vi "test_PhotonPoseEstimator_ClosestToLastfPose.vi"(8 "error in (no error)":errorcluster) -> (0 "error out":errorcluster, 3 "Test Passed":bool)   [LabVIEW 2019]
uses:
  <vilib>/Rock Robotics/WPI/ThirdParty/PhotonVisionLib/TypeDef/PhotonEstimatedRobotPoseType.ctl
  <vilib>/Rock Robotics/WPI/ThirdParty/JAS_Junk/TrajLib/TypeDef/POSE3D.ctl
  <vilib>/Rock Robotics/WPI/ThirdParty/JAS_Junk/TrajLib/TypeDef/TRANSLATION3D.ctl
  <vilib>/Rock Robotics/WPI/ThirdParty/JAS_Junk/TrajLib/TypeDef/ROTATION3D.ctl
  <vilib>/Rock Robotics/WPI/ThirdParty/JAS_Junk/TrajLib/TypeDef/QUATERNION.ctl
  <vilib>/Rock Robotics/WPI/ThirdParty/PhotonVisionLib/TypeDef/PhotonTrackedTargetType.ctl
  <vilib>/Rock Robotics/WPI/ThirdParty/PhotonVisionLib/TypeDef/TargetCornerType.ctl
  <vilib>/Rock Robotics/WPI/ThirdParty/JAS_Junk/TrajLib/TypeDef/TRANSFORM3D.ctl
  <vilib>/Rock Robotics/WPI/ThirdParty/PhotonVisionLib/Enum/PhotonPoseStrategy_ENUM.ctl
  <vilib>/Rock Robotics/WPI/ThirdParty/JAS_Junk/TrajLib/VI/Quaternion_New.vi
  <vilib>/Rock Robotics/WPI/ThirdParty/PhotonVisionLib/SubVI/PhotonTargetModel_New_AprilTag36H11.vi
  <vilib>/Rock Robotics/WPI/ThirdParty/JAS_Junk/TrajLib/VI/TimeInterpRotation2d_New.vi
  <vilib>/Rock Robotics/WPI/ThirdParty/JAS_Junk/TrajLib/VI/Transform3d_Equals.vi
  <vilib>/Rock Robotics/WPI/ThirdParty/PhotonVisionLib/SubVI/PhotonPoseEstimator_SetCamera.vi
  <vilib>/Rock Robotics/WPI/ThirdParty/PhotonVisionLib/SubVI/PhotonPoseEstimator_SetRobotToCameraTransform.vi
  <vilib>/Rock Robotics/WPI/ThirdParty/PhotonVisionLib/SubVI/PhotonEstimatedRobotPose_GetAll.vi
  <vilib>/Rock Robotics/WPI/ThirdParty/JAS_Junk/TrajLib/VI/Pose3d_ToPose2d.vi
  <vilib>/Rock Robotics/WPI/ThirdParty/PhotonVisionLib/SubVI/PhotonPoseEstimator_Update_All.vi
  <vilib>/Rock Robotics/WPI/ThirdParty/PhotonVisionLib/SubVI/PhotonPoseEstimator_GetEmptyPose.vi
  <vilib>/Rock Robotics/WPI/ThirdParty/PhotonVisionLib/SubVI/PhotonPoseEstimator_EstimateClosestToLastPose.vi
  <vilib>/Rock Robotics/WPI/ThirdParty/PhotonVisionLib/SubVI/PhotonPoseEstimator_GetLastPose.vi
  <vilib>/Rock Robotics/WPI/ThirdParty/PhotonVisionLib/SubVI/PhotonPipelineResult_GetTimeStampSecs.vi
  <vilib>/Rock Robotics/WPI/ThirdParty/PhotonVisionLib/SubVI/PhotonTargetModel_New_RectPlanar.vi
  <vilib>/Rock Robotics/WPI/ThirdParty/JAS_Junk/TrajLib/Conv_Inches_Meters.vi
  <vilib>/Rock Robotics/WPI/ThirdParty/JAS_Junk/TrajLib/VI/Transform3d_GetTranslation3d.vi
  <vilib>/Rock Robotics/WPI/ThirdParty/JAS_Junk/TrajLib/VI/Transform3d_GetRotation3d.vi
  <vilib>/Rock Robotics/WPI/ThirdParty/JAS_Junk/TrajLib/VI/Rotation3d_Equals.vi
  <vilib>/Rock Robotics/WPI/ThirdParty/JAS_Junk/TrajLib/VI/Translation3d_Equals.vi
  <vilib>/Rock Robotics/WPI/ThirdParty/JAS_Junk/TrajLib/VI/Pose3d_getTranslation3d.vi
  <vilib>/Rock Robotics/WPI/ThirdParty/JAS_Junk/TrajLib/VI/Pose3d_getRotation3d.vi
  <vilib>/Rock Robotics/WPI/ThirdParty/JAS_Junk/TrajLib/VI/Translation3d_ToTranslation2d.vi
  <vilib>/Rock Robotics/WPI/ThirdParty/JAS_Junk/TrajLib/VI/Rotation3d_ToRotation2d.vi
  <vilib>/Rock Robotics/WPI/ThirdParty/JAS_Junk/TrajLib/Pose2d_New_TRRO.vi
  <vilib>/Rock Robotics/WPI/ThirdParty/PhotonVisionLib/SubVI/PhotonPoseEstimator_EstimateLowestAmbiguityPose.vi
  <vilib>/Rock Robotics/WPI/ThirdParty/PhotonVisionLib/SubVI/PhotonPoseEstimator_EstimateClosestToCameraHeightPose.vi
  <vilib>/Rock Robotics/WPI/ThirdParty/PhotonVisionLib/SubVI/PhotonPoseEstimator_EstimateClosestToReferencePose.vi
  <vilib>/Rock Robotics/WPI/ThirdParty/PhotonVisionLib/SubVI/PhotonPoseEstimator_GetReferencePose.vi
  <vilib>/Rock Robotics/WPI/ThirdParty/PhotonVisionLib/SubVI/PhotonPoseEstimator_SetReferencePose.vi
  <vilib>/Rock Robotics/WPI/ThirdParty/PhotonVisionLib/SubVI/PhotonPoseEstimator_EstimateAverageBestTargetsPose.vi
  <vilib>/Rock Robotics/WPI/ThirdParty/PhotonVisionLib/SubVI/PhotonPoseEstimator_EstimateMultiTagOnCoprocPose.vi
  <vilib>/Rock Robotics/WPI/ThirdParty/PhotonVisionLib/SubVI/PhotonPoseEstimator_EstimatePnpDistanceTrigSolvePose.vi
  <vilib>/Rock Robotics/WPI/ThirdParty/PhotonVisionLib/SubVI/PhotonPoseEstimator_Strategy_constrainedPnpStrategy.vi
  <vilib>/Rock Robotics/WPI/ThirdParty/JAS_Junk/TrajLib/VI/Rotation3d_Create_AxisAngle.vi
  <vilib>/Rock Robotics/WPI/ThirdParty/JAS_Junk/TrajLib/VI/Pose3d_New.vi
  <vilib>/Rock Robotics/WPI/ThirdParty/PhotonVisionLib/SubVI/PhotonPipelineResult_HasTargets.vi
  <vilib>/Rock Robotics/WPI/ThirdParty/PhotonVisionLib/SubVI/PhotonEstimatedRobotPose_New.vi
  <vilib>/Rock Robotics/WPI/ThirdParty/PhotonVisionLib/SubVI/PhotonPipelineResult_GetTargets.vi
  <vilib>/Rock Robotics/WPI/ThirdParty/JAS_Junk/TrajLib/VI/AprilTagFieldLayout_GetTagPose.vi
  <vilib>/Rock Robotics/WPI/ThirdParty/PhotonVisionLib/SubVI/PhotonTrackedTarget_GetFiducialId.vi
  <vilib>/Rock Robotics/WPI/ThirdParty/PhotonVisionLib/SubVI/PhotonTrackedTarget_GetAltCameraToTarget.vi
  <vilib>/Rock Robotics/WPI/ThirdParty/PhotonVisionLib/SubVI/PhotonTrackedTarget_GetBestCameraToTarget.vi
  <vilib>/Rock Robotics/WPI/ThirdParty/PhotonVisionLib/SubVI/PhotonPoseEstimator_Strategy_closestToReferencePose_calc.vi
  <vilib>/Rock Robotics/WPI/ThirdParty/PhotonVisionLib/SubVI/PhotonTrackedTarget_GetPoseAmbiguity.vi
  <vilib>/Rock Robotics/WPI/ThirdParty/PhotonVisionLib/SubVI/PhotonPoseEstimator_GetFieldTags.vi
  <vilib>/Rock Robotics/WPI/ThirdParty/PhotonVisionLib/SubVI/PhotonPoseEstimator_GetRobotToCameraTransform.vi
  <vilib>/Rock Robotics/WPI/ThirdParty/PhotonVisionLib/SubVI/PhotonPoseEstimator_GetHighestAmbiguity.vi
  <vilib>/Rock Robotics/WPI/ThirdParty/PhotonVisionLib/SubVI/PhotonTargetModel_New.vi
  <vilib>/Rock Robotics/WPI/ThirdParty/JAS_Junk/TrajLib/VI/Rotation3d_GetQuaterion.vi
  <vilib>/Rock Robotics/WPI/ThirdParty/JAS_Junk/TrajLib/VI/Quaternion_Equals.vi
  <vilib>/Rock Robotics/WPI/ThirdParty/JAS_Junk/TrajLib/Translation2d_Create.vi
  <vilib>/Rock Robotics/WPI/ThirdParty/JAS_Junk/TrajLib/Rotation2d_CreateAngle.vi
  <vilib>/Rock Robotics/WPI/ThirdParty/JAS_Junk/TrajLib/VI/Rotation3d_GetXYZ.vi
  <vilib>/Rock Robotics/WPI/ThirdParty/JAS_Junk/TrajLib/VI/Pose3d_TransformBy.vi
  <vilib>/Rock Robotics/WPI/ThirdParty/JAS_Junk/TrajLib/VI/Transform3d_Inverse.vi
  <vilib>/Rock Robotics/WPI/ThirdParty/PhotonVisionLib/SubVI/PhotonPoseEstimator_Strategy_closestToCameraHeight_calc.vi
  <vilib>/Rock Robotics/WPI/ThirdParty/PhotonVisionLib/SubVI/PhotonPoseEstimator_Strategy_averageBestTargets_calc.vi
  <vilib>/Rock Robotics/WPI/ThirdParty/JAS_Junk/TrajLib/VI/Rotation3d_Plus.vi
  <vilib>/Rock Robotics/WPI/ThirdParty/JAS_Junk/TrajLib/VI/Translation3d_Plus.vi
  <vilib>/Rock Robotics/WPI/ThirdParty/JAS_Junk/TrajLib/VI/Translation3d_Times.vi
  <vilib>/Rock Robotics/WPI/ThirdParty/JAS_Junk/TrajLib/VI/Rotation3d_Times.vi
  <vilib>/Rock Robotics/WPI/ThirdParty/JAS_Junk/TrajLib/VI/Rotation3d_Create_Default.vi
  <vilib>/Rock Robotics/WPI/ThirdParty/JAS_Junk/TrajLib/VI/Translation3d_Create_Default.vi
  <vilib>/Rock Robotics/WPI/ThirdParty/JAS_Junk/TrajLib/VI/Pose3d_New_Default.vi
  <vilib>/Rock Robotics/WPI/ThirdParty/JAS_Junk/TrajLib/VI/Pose3d_Plus.vi
  <vilib>/Rock Robotics/WPI/ThirdParty/JAS_Junk/TrajLib/VI/Pose3d_RelativeTo.vi
  <vilib>/Rock Robotics/WPI/ThirdParty/JAS_Junk/TrajLib/VI/AprilTagFieldLayout_GetOriginPosition.vi
  <vilib>/Rock Robotics/WPI/ThirdParty/PhotonVisionLib/SubVI/PhotonPipelineResult_GetMultiTagResult.vi
  <vilib>/Rock Robotics/WPI/ThirdParty/PhotonVisionLib/SubVI/PhotonPipelineResult_GetBestTarget.vi
  <vilib>/Rock Robotics/WPI/ThirdParty/PhotonVisionLib/SubVI/PhotonTrackedTarget_GetPitch.vi
  <vilib>/Rock Robotics/WPI/ThirdParty/PhotonVisionLib/SubVI/PhotonTrackedTarget_GetYaw.vi
  <vilib>/Rock Robotics/WPI/ThirdParty/JAS_Junk/TrajLib/Units_DegreesToRadians.vi
  <vilib>/Rock Robotics/WPI/ThirdParty/JAS_Junk/TrajLib/VI/Translation3d_GetNorm.vi
  <vilib>/Rock Robotics/WPI/ThirdParty/JAS_Junk/TrajLib/VI/Translation3d_Create_DistAng.vi
  <vilib>/Rock Robotics/WPI/ThirdParty/JAS_Junk/TrajLib/VI/Translation3d_RotateBy.vi
  <vilib>/Rock Robotics/WPI/ThirdParty/JAS_Junk/TrajLib/Translation2d_RotateBy.vi
  <vilib>/Rock Robotics/WPI/ThirdParty/JAS_Junk/TrajLib/Pose2d_getTranslation.vi
  <vilib>/Rock Robotics/WPI/ThirdParty/JAS_Junk/TrajLib/Translation2d_Plus.vi
  <vilib>/Rock Robotics/WPI/ThirdParty/JAS_Junk/TrajLib/Translation2d_UnaryMinus.vi
  <vilib>/Rock Robotics/WPI/ThirdParty/JAS_Junk/TrajLib/VI/Pose3d_New_Pose2d.vi
  <vilib>/Rock Robotics/WPI/ThirdParty/JAS_Junk/TrajLib/VI/TimeInterpRotation2d_GetSample.vi
  <vilib>/Rock Robotics/WPI/ThirdParty/PhotonVisionLib/SubVI/PhotonPoseEstimator_GetHeadingBuffer.vi
  <vilib>/Rock Robotics/WPI/ThirdParty/JAS_Junk/TrajLib/VI/Vector_Norm.vi
  <vilib>/Rock Robotics/WPI/ThirdParty/JAS_Junk/TrajLib/VecBuilder_ArrayBy1Fill.vi
  <vilib>/Rock Robotics/WPI/ThirdParty/JAS_Junk/TrajLib/VI/AprilTag_GetAll.vi
  <vilib>/Rock Robotics/WPI/ThirdParty/JAS_Junk/TrajLib/Transform2d_Create_TransRot.vi
  <vilib>/Rock Robotics/WPI/ThirdParty/PhotonVisionLib/SubVI/PhotonPoseEstimator_CalcDifference.vi
  <vilib>/Rock Robotics/WPI/ThirdParty/JAS_Junk/TrajLib/VI/Quaternion_Get_Vect.vi
  <vilib>/Rock Robotics/WPI/ThirdParty/JAS_Junk/TrajLib/VI/Quaternion_Get_W.vi
  <vilib>/Rock Robotics/WPI/ThirdParty/JAS_Junk/TrajLib/VI/Quaternion_Get_All.vi
  <vilib>/Rock Robotics/WPI/ThirdParty/JAS_Junk/TrajLib/VI/Rotation3d_UnaryMinus.vi
  <vilib>/Rock Robotics/WPI/ThirdParty/JAS_Junk/TrajLib/VI/Translation3d_UnaryMinus.vi
  <vilib>/Rock Robotics/WPI/ThirdParty/JAS_Junk/TrajLib/VI/Transform3d_GetXYZ.vi
  <vilib>/Rock Robotics/WPI/ThirdParty/JAS_Junk/TrajLib/VI/Pose3d_getXYZ.vi
  <vilib>/Rock Robotics/WPI/ThirdParty/JAS_Junk/TrajLib/VI/Rotation3d_RotateBy.vi
  <vilib>/Rock Robotics/WPI/ThirdParty/JAS_Junk/TrajLib/VI/Translation3d_GetXYZ.vi
  <vilib>/Rock Robotics/WPI/ThirdParty/JAS_Junk/TrajLib/VI/Quaternion_New_Default.vi
  <vilib>/Rock Robotics/WPI/ThirdParty/JAS_Junk/TrajLib/VI/Transform3d_Create_Pose3dPose3d.vi
  <vilib>/Rock Robotics/WPI/ThirdParty/JAS_Junk/TrajLib/Conv_Deg_Radians.vi
  <vilib>/Rock Robotics/WPI/ThirdParty/JAS_Junk/TrajLib/VI/Quaternion_Times.vi
  <vilib>/Rock Robotics/WPI/ThirdParty/JAS_Junk/TrajLib/VI/Quaternion_Inverse.vi
  <vilib>/Rock Robotics/WPI/ThirdParty/JAS_Junk/TrajLib/Pose2d_getXYAngle.vi
  <vilib>/Rock Robotics/WPI/ThirdParty/JAS_Junk/TrajLib/Rotation2d_Interpolate.vi
  <vilib>/Rock Robotics/WPI/ThirdParty/JAS_Junk/TrajLib/MatBuilder_Create.vi
  <vilib>/Rock Robotics/WPI/ThirdParty/JAS_Junk/TrajLib/VI/Translation3d_GetDistance.vi
  <vilib>/Rock Robotics/WPI/ThirdParty/JAS_Junk/TrajLib/VI/Rotation3d_Create_Quaternion.vi
  <vilib>/Rock Robotics/WPI/ThirdParty/JAS_Junk/TrajLib/VI/Translation3d_Minus.vi
  <vilib>/Rock Robotics/WPI/ThirdParty/JAS_Junk/TrajLib/VI/Rotation3d_Minus.vi
  <vilib>/Rock Robotics/WPI/ThirdParty/JAS_Junk/TrajLib/Rotation2d_Plus.vi
  <vilib>/Rock Robotics/WPI/ThirdParty/JAS_Junk/TrajLib/Rotation2d_Minus.vi
  <vilib>/Rock Robotics/WPI/ThirdParty/JAS_Junk/TrajLib/MathUtil_Clamp.vi
  <vilib>/Rock Robotics/WPI/ThirdParty/JAS_Junk/TrajLib/Rotation2d_Times.vi
  <vilib>/Rock Robotics/WPI/ThirdParty/JAS_Junk/TrajLib/VI/Quaternion_Normalize.vi
  <vilib>/Rock Robotics/WPI/ThirdParty/JAS_Junk/TrajLib/Rotation2d_RotateBy.vi
  <vilib>/Rock Robotics/WPI/ThirdParty/JAS_Junk/TrajLib/Rotation2d_UnaryMinus.vi
  <vilib>/Rock Robotics/WPI/ThirdParty/JAS_Junk/TrajLib/Rotation2d_CreateXY.vi
  <vilib>/Rock Robotics/WPI/ThirdParty/JAS_Junk/TrajLib/Util_CalcDist.vi
  <vilib>/Rock Robotics/WPI/ThirdParty/PhotonVisionLib/SubVI/PhotonVision_Globals.vi
  <vilib>/gmath/interp.llb/Search Ordered Table.vi
  <vilib>/Rock Robotics/WPI/ThirdParty/JAS_Junk/TrajLib/Trajectory_Library.lvlib
  <vilib>/Rock Robotics/WPI/ThirdParty/PhotonVisionLib/PhotonVisionLib.lvlib
panel:
  out "Test 2 Passed":bool
  out "Test 1 Passed":bool
  out "2nd Pos Found":bool
  out "2nd Pose Est":T1={"EstimatedPose"={"Translation3d"={"X"=0.0, "Y"=0.0, "Z"=0.0}, "Rotation3d"={"Q_quaternion"={"R"=1.0, "V"=[0.0, 0.0, 0.0]}}}, "TimeStamp_Seconds"=0.0, "targetsUsed"=[], "Strategy"=enum."LOWEST_AMBIGUITY"} {"targetsUsed"."AltCameraToTarget"."TRANSLATION3D"."Z" format="%14.3f"; "targetsUsed"."AltCameraToTarget"."TRANSLATION3D"."Y" format="%14.3f"; "targetsUsed"."AltCameraToTarget"."TRANSLATION3D"."X" format="%14.3f"; "targetsUsed"."BestCameraToTarget"."TRANSLATION3D"."Z" format="%14.3f"; "targetsUsed"."BestCameraToTarget"."TRANSLATION3D"."Y" format="%14.3f"; "targetsUsed"."BestCameraToTarget"."TRANSLATION3D"."X" format="%14.3f"; "EstimatedPose"."Translation3d"."Z" format="%14.3f"; "EstimatedPose"."Translation3d"."Y" format="%14.3f"; "EstimatedPose"."Translation3d"."X" format="%14.3f"}
  out "1st Pos Found":bool
  out "1st Pose Est":T1={"EstimatedPose"={"Translation3d"={"X"=0.0, "Y"=0.0, "Z"=0.0}, "Rotation3d"={"Q_quaternion"={"R"=1.0, "V"=[0.0, 0.0, 0.0]}}}, "TimeStamp_Seconds"=0.0, "targetsUsed"=[], "Strategy"=enum."LOWEST_AMBIGUITY"} {"targetsUsed"."AltCameraToTarget"."TRANSLATION3D"."Z" format="%14.3f"; "targetsUsed"."AltCameraToTarget"."TRANSLATION3D"."Y" format="%14.3f"; "targetsUsed"."AltCameraToTarget"."TRANSLATION3D"."X" format="%14.3f"; "targetsUsed"."BestCameraToTarget"."TRANSLATION3D"."Z" format="%14.3f"; "targetsUsed"."BestCameraToTarget"."TRANSLATION3D"."Y" format="%14.3f"; "targetsUsed"."BestCameraToTarget"."TRANSLATION3D"."X" format="%14.3f"; "EstimatedPose"."Translation3d"."Z" format="%14.3f"; "EstimatedPose"."Translation3d"."Y" format="%14.3f"; "EstimatedPose"."Translation3d"."X" format="%14.3f"}
  out "Test 0 Passed":bool
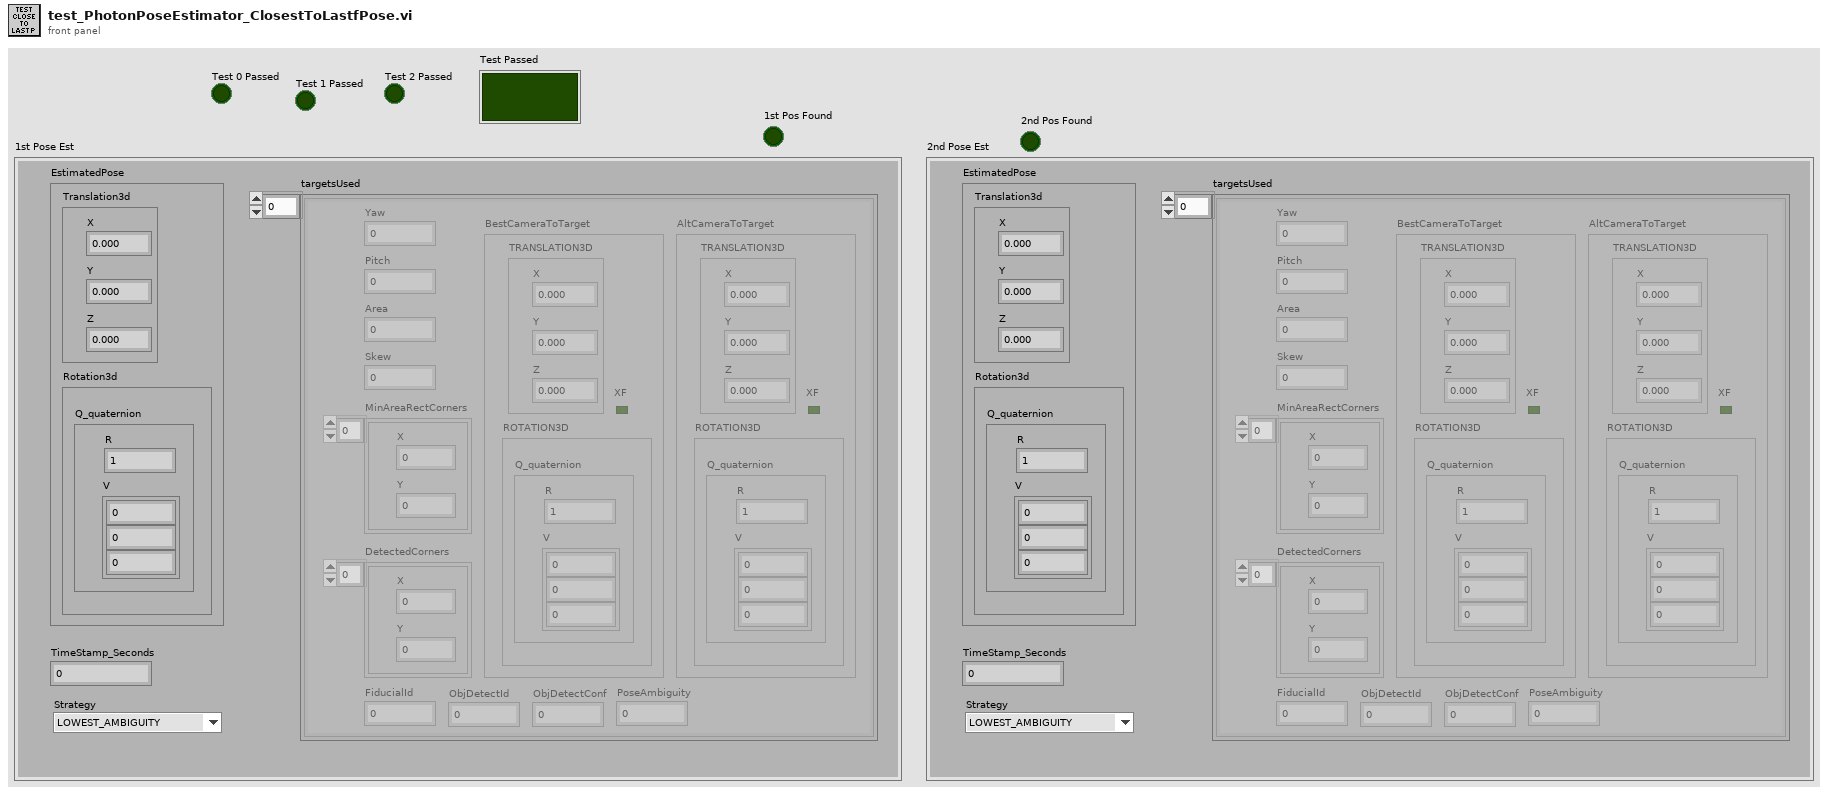
[diagram p1: front panel]
types:
  T1 = typedef "PhotonVisionLib.lvlib/PhotonEstimatedRobotPoseType.ctl" = cluster{"EstimatedPose":T2, "TimeStamp_Seconds":dbl, "targetsUsed":T6[], "Strategy":T9}
  T2 = typedef "Trajectory_Library.lvlib/POSE3D.ctl" = cluster{"Translation3d":T3, "Rotation3d":T4}
  T3 = typedef "Trajectory_Library.lvlib/TRANSLATION3D.ctl" = cluster{"X":dbl, "Y":dbl, "Z":dbl}
  T4 = typedef "Trajectory_Library.lvlib/ROTATION3D.ctl" = cluster{"Q_quaternion":T5}
  T5 = typedef "Trajectory_Library.lvlib/QUATERNION.ctl" = cluster{"R":dbl, "V":dbl[]}
  T6 = typedef "PhotonVisionLib.lvlib/PhotonTrackedTargetType.ctl" = cluster{"Yaw":dbl, "Pitch":dbl, "Area":dbl, "Skew":dbl, "MinAreaRectCorners":T7[], "BestCameraToTarget":T8, "FiducialId":i32, "AltCameraToTarget":T8, "PoseAmbiguity":dbl, "DetectedCorners":T7[], "ObjDetectId":i32, "ObjDetectConf":sgl}
  T7 = typedef "PhotonVisionLib.lvlib/TargetCornerType.ctl" = cluster{"X":dbl, "Y":dbl}
  T8 = typedef "Trajectory_Library.lvlib/TRANSFORM3D.ctl" = cluster{"TRANSLATION3D":T3, "ROTATION3D":T4, "XF":bool}
  T9 = typedef "PhotonVisionLib.lvlib/PhotonPoseStrategy_ENUM.ctl" = enum16{"LOWEST_AMBIGUITY", "CLOSEST_TO_CAMERA_HEIGHT", "CLOSEST_TO_REFERENCE_POSE", "CLOSEST_TO_LAST_POSE", "AVERAGE_BEST_TARGETS", "MULTI_TAG_PNP_ON_COPROCESSOR", "MULTI_TAG_PNP_ON_RIO", "PNP_DISTANCE_TRIG_SOLVE", "CONSTRAINED_SOLVEPNP"}
  T10 = typedef "Trajectory_Library.lvlib/AprilTagFieldLayout.ctl" = cluster{"AprilTagMap":map{i32, T11}, "FieldLength":dbl, "FieldWidth":dbl, "OriginPosition ":T12, "OriginPose3d":T2}
  T11 = typedef "Trajectory_Library.lvlib/AprilTag.ctl" = cluster{"ID":i32, "POSE3D":T2}
  T12 = typedef "Trajectory_Library.lvlib/AprilTagFieldLayoutOrignPosition_ENUM.ctl" = enum16{"kBlueAllianceWallRightSide,", "kRedAllianceWallRightSide,"}
  T13 = typedef "PhotonVisionLib.lvlib/PhotonPipelineMetadataType.ctl" = cluster{"CaptureTimestampMicros":i64, "PublishTimestampMicros":i64, "SequenceID":i64, "TimeSinceLastPong":i64}
  T14 = typedef "PhotonVisionLib.lvlib/PhotonPipelineResultType.ctl" = cluster{"Targets":T6[], "PhotonMultiTargetPNPResult":T15, "PhotonPipelineMetadata":T13}
  T15 = typedef "PhotonVisionLib.lvlib/PhotonMultiTargetPNPResultType.ctl" = cluster{"PhotonPNPResult":T16, "FiducialIDsUsed":i16[]}
  T16 = typedef "PhotonVisionLib.lvlib/PhotonPNPResultType.ctl" = cluster{"IsPresent":bool, "bestReprojErr":dbl, "altReprojErr":dbl, "ambiguity":dbl, "Best":T8, "Alt":T8}
  T17 = typedef "PhotonVisionLib.lvlib/PhotonPoseEstimatorType.ctl" = cluster{"LastPose":T2, "ReferencePose":T2, "FieldTags":T10, "PrimaryStratety":T9, "Camera":string, "RobotToCamera":T8, "ReportedErrors":dbl[], "HighestAmbiguity":dbl, "MultiTagFallbackStrategy":T9, "PoseCacheTimeoutSec":dbl, "PhotonTargetModel":T18, "BaseNTName":string}
  T18 = typedef "PhotonVisionLib.lvlib/PhotonTargetModel.ctl" = cluster{"Vertices":T3[], "IsPlaner":bool, "IsSpherical":bool}
  T19 = typedef "PhotonVisionLib.lvlib/PhotonPoseEstimator_Configuration.ctl" = cluster{"Primary Strategy":T9, "Camera":string, "Initial Pose":T2, "HighestAmbiguity":dbl, "RobotToCamera":T8, "FallBack Strategy":T9, "BaseNTName":string}
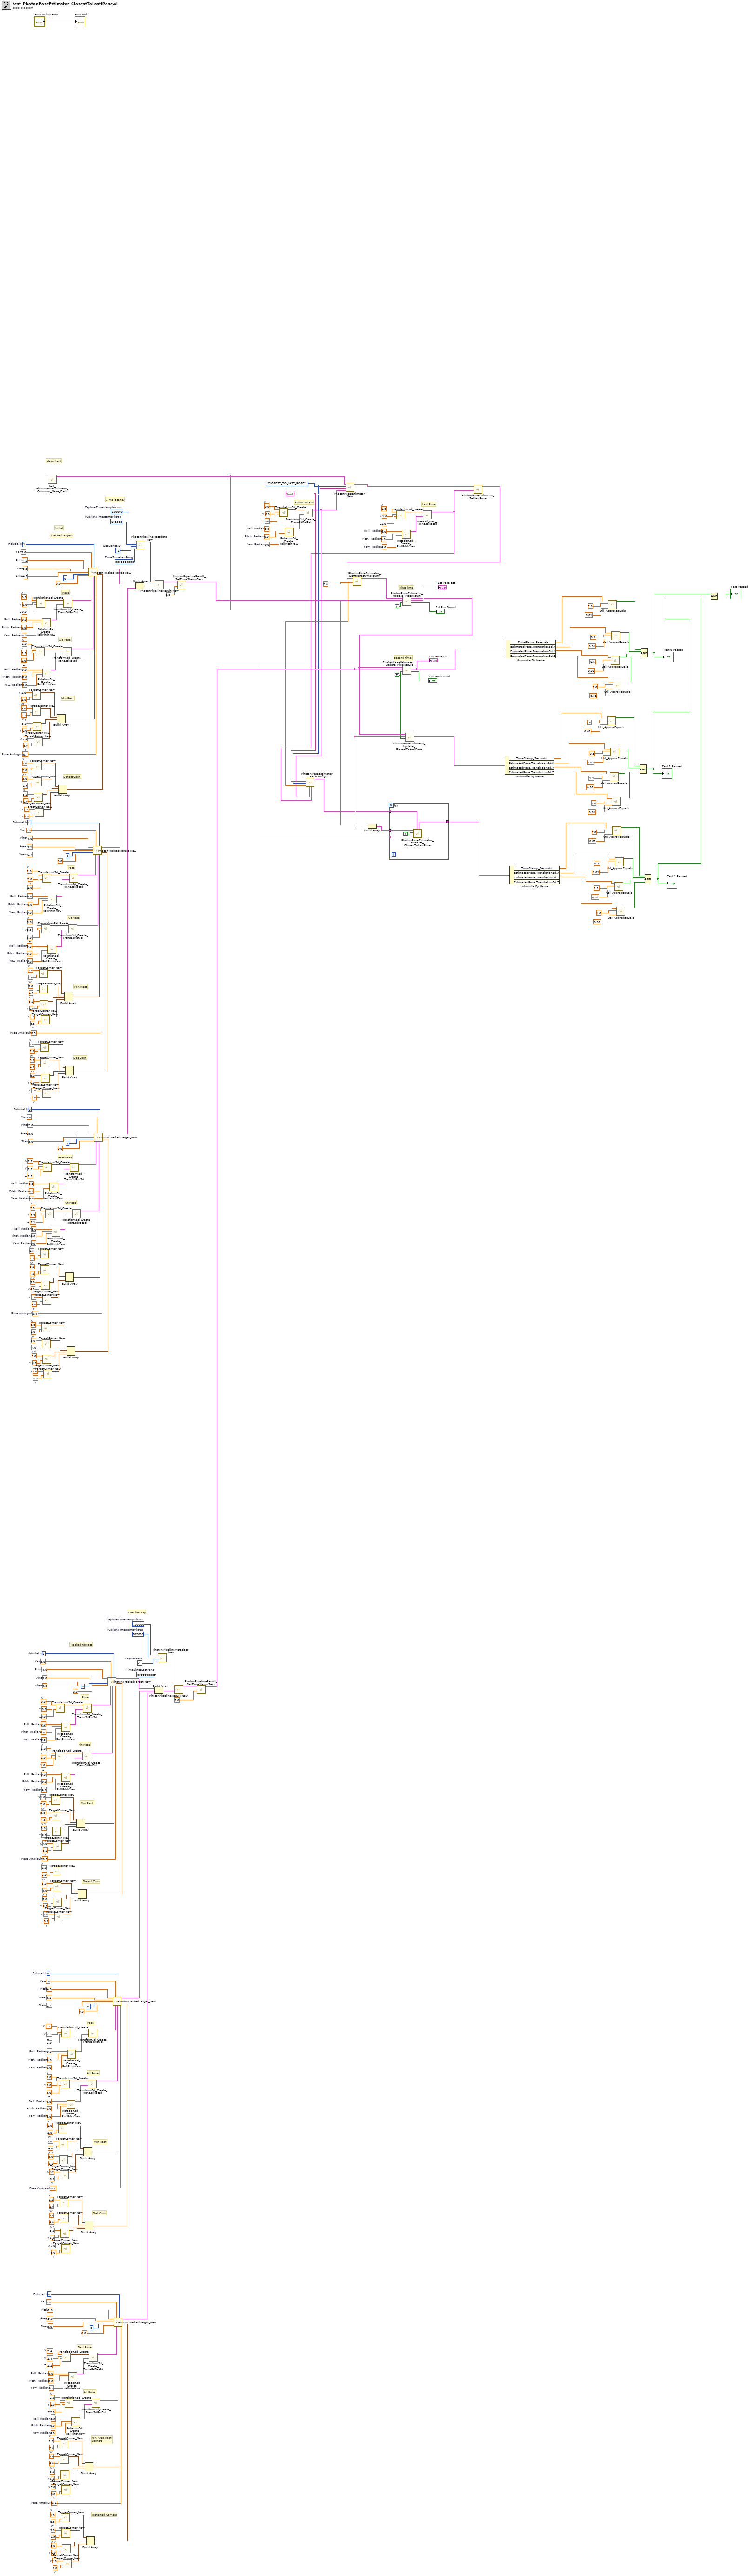
[diagram p0: block diagram]
diagram:
  w6 = 2.0 ("HighestAmbiguity")
  w65 = i64 100000  # CaptureTimestampMicros
  w66 = i64 102000  # PublishTimestampMicros
  w67 = i64 -1  # SequenceID
  w68 = i64 9999999999  # TimeSinceLastPong
  w70 = i64 100000  # CaptureTimestampMicros
  w71 = i64 102000  # PublishTimestampMicros
  w72 = i64 -1  # SequenceID
  w73 = i64 9999999999  # TimeSinceLastPong
  w47 = TRUE ("Has Results")
  w91 = 0.0  # Roll  Radians
  w90 = 0.0  # Pitch  Radians
  w89 = 0.0  # Yaw  Radians
  w94 = 2.2  # Z
  w93 = 2.4  # X
  w92 = 2.4  # Y
  w99 = 0.0  # Roll  Radians
  w98 = 0.0  # Pitch  Radians
  w97 = 0.0  # Yaw  Radians
  w102 = 2.0  # Z
  w101 = 2.0  # X
  w100 = 1.0  # Y
  w109 = 7.0  # X
  w110 = 8.0  # Y
  w111 = 5.0  # X
  w112 = 6.0  # Y
  w113 = 3.0  # X
  w114 = 4.0  # Y
  w115 = 1.0  # X
  w116 = 2.0  # Y
  w121 = 7.0  # X
  w122 = 8.0  # Y
  w123 = 5.0  # X
  w124 = 6.0  # Y
  w125 = 3.0  # X
  w126 = 4.0  # Y
  w127 = 1.0  # X
  w128 = 2.0  # Y
  w129 = -2.0  # Pitch
  w130 = 19.0  # Area
  w131 = 3.0  # Skew
  w132 = 0  # Fiducial Id
  w133 = 0.4  # Pose Ambiguity
  w134 = 9.0  # Yaw
  w141 = 0.0  # Roll  Radians
  w140 = 0.0  # Pitch  Radians
  w139 = 0.0  # Yaw  Radians
  w144 = 2.0  # Z
  w143 = 2.1  # X
  w142 = 1.9  # Y
  w149 = 0.0  # Roll  Radians
  w148 = 0.0  # Pitch  Radians
  w147 = 0.0  # Yaw  Radians
  w152 = 3.0  # Z
  w151 = 3.0  # X
  w150 = 3.0  # Y
  w159 = 7.0  # X
  w160 = 8.0  # Y
  w161 = 5.0  # X
  w162 = 6.0  # Y
  w163 = 3.0  # X
  w164 = 4.0  # Y
  w165 = 1.0  # X
  w166 = 2.0  # Y
  w171 = 7.0  # X
  w172 = 8.0  # Y
  w173 = 5.0  # X
  w174 = 6.0  # Y
  w175 = 3.0  # X
  w176 = 4.0  # Y
  w177 = 1.0  # X
  w178 = 2.0  # Y
  w179 = -4.0  # Pitch
  w180 = 9.1  # Area
  w181 = 6.7  # Skew
  w182 = 0  # Fiducial Id
  w183 = 0.3  # Pose Ambiguity
  w184 = 3.0  # Yaw
  w190 = 0.0  # Roll  Radians
  w189 = 0.0  # Pitch  Radians
  w188 = 0.0  # Yaw  Radians
  w193 = 0.0  # Z
  w192 = 0.0  # X
  w191 = 0.0  # Y
  w198 = 0.0  # Roll  Radians
  w197 = 0.0  # Pitch  Radians
  w196 = 0.0  # Yaw  Radians
  w201 = 1.0  # Z
  w200 = 1.0  # X
  w199 = 1.0  # Y
  w208 = 7.0  # X
  w209 = 8.0  # Y
  w210 = 5.0  # X
  w211 = 6.0  # Y
  w212 = 3.0  # X
  w213 = 4.0  # Y
  w214 = 1.0  # X
  w215 = 2.0  # Y
  w220 = 7.0  # X
  w221 = 8.0  # Y
  w222 = 5.0  # X
  w223 = 6.0  # Y
  w224 = 3.0  # X
  w225 = 4.0  # Y
  w226 = 1.0  # X
  w227 = 2.0  # Y
  w228 = -4.0  # Pitch
  w229 = 9.0  # Area
  w230 = 4.0  # Skew
  w231 = 1  # Fiducial Id
  w232 = 0.7  # Pose Ambiguity
  w233 = 3.0  # Yaw
  w238 = 0.0  # Roll  Radians
  w237 = 0.0  # Pitch  Radians
  w236 = 0.0  # Yaw  Radians
  w241 = 1.0  # Z
  w240 = 1.0  # X
  w239 = 1.0  # Y
  w251 = 0.0  # Roll  Radians
  w250 = 0.0  # Pitch  Radians
  w249 = 0.0  # Yaw  Radians
  w254 = 0.0  # Z
  w253 = 0.0  # X
  w252 = 0.0  # Y
  w5 = "Junk" ("Camera")
  w4 = PhotonPoseStrategy_ENUM."CLOSEST_TO_LAST_POSE" ("Strategy")
  w276 = 0.0  # Roll  Radians
  w275 = 0.0  # Pitch  Radians
  w274 = 0.0  # Yaw  Radians
  w279 = 2.2  # Z
  w278 = 2.2  # X
  w277 = 2.2  # Y
  w284 = 0.0  # Roll  Radians
  w283 = 0.0  # Pitch  Radians
  w282 = 0.0  # Yaw  Radians
  w287 = 2.1  # Z
  w286 = 2.0  # X
  w285 = 1.9  # Y
  w294 = 7.0  # X
  w295 = 8.0  # Y
  w296 = 5.0  # X
  w297 = 6.0  # Y
  w298 = 3.0  # X
  w299 = 4.0  # Y
  w300 = 1.0  # X
  w301 = 2.0  # Y
  w306 = 7.0  # X
  w307 = 8.0  # Y
  w308 = 5.0  # X
  w309 = 6.0  # Y
  w310 = 3.0  # X
  w311 = 4.0  # Y
  w312 = 1.0  # X
  w313 = 2.0  # Y
  w314 = -2.0  # Pitch
  w315 = 19.0  # Area
  w316 = 3.0  # Skew
  w317 = 0  # Fiducial Id
  w318 = 0.4  # Pose Ambiguity
  w319 = 9.0  # Yaw
  w326 = 0.0  # Roll  Radians
  w325 = 0.0  # Pitch  Radians
  w324 = 0.0  # Yaw  Radians
  w329 = 2.0  # Z
  w328 = 2.0  # X
  w327 = 2.0  # Y
  w334 = 0.0  # Roll  Radians
  w333 = 0.0  # Pitch  Radians
  w332 = 0.0  # Yaw  Radians
  w337 = 3.0  # Z
  w336 = 3.0  # X
  w335 = 3.0  # Y
  w344 = 7.0  # X
  w345 = 8.0  # Y
  w346 = 5.0  # X
  w347 = 6.0  # Y
  w348 = 3.0  # X
  w349 = 4.0  # Y
  w350 = 1.0  # X
  w351 = 2.0  # Y
  w356 = 7.0  # X
  w357 = 8.0  # Y
  w358 = 5.0  # X
  w359 = 6.0  # Y
  w360 = 3.0  # X
  w361 = 4.0  # Y
  w362 = 1.0  # X
  w363 = 2.0  # Y
  w364 = -4.0  # Pitch
  w365 = 9.1  # Area
  w366 = 6.7  # Skew
  w367 = 1  # Fiducial Id
  w368 = 0.3  # Pose Ambiguity
  w369 = 3.0  # Yaw
  w376 = 0.0  # Roll  Radians
  w375 = 0.0  # Pitch  Radians
  w374 = 0.0  # Yaw  Radians
  w379 = 0.0  # Z
  w378 = 0.0  # X
  w377 = 0.0  # Y
  w384 = 0.0  # Roll  Radians
  w383 = 0.0  # Pitch  Radians
  w382 = 0.0  # Yaw  Radians
  w387 = 1.0  # Z
  w386 = 1.0  # X
  w385 = 1.0  # Y
  w394 = 7.0  # X
  w395 = 8.0  # Y
  w396 = 5.0  # X
  w397 = 6.0  # Y
  w398 = 3.0  # X
  w399 = 4.0  # Y
  w400 = 1.0  # X
  w401 = 2.0  # Y
  w406 = 7.0  # X
  w407 = 8.0  # Y
  w408 = 5.0  # X
  w409 = 6.0  # Y
  w410 = 3.0  # X
  w411 = 4.0  # Y
  w412 = 1.0  # X
  w413 = 2.0  # Y
  w414 = -4.0  # Pitch
  w415 = 9.0  # Area
  w416 = 4.0  # Skew
  w417 = 1  # Fiducial Id
  w418 = 0.7  # Pose Ambiguity
  w419 = 3.0  # Yaw
  # "2 ms latency"
  # "2 ms latency"
  # "Min Area Rect\nCorners"
  # "Detected Corners"
  # "second time"
  # "First time"
  # "Initial"
  # "Det Corn"
  # "Min Rect"
  # "Pose"
  # "Detect Corn"
  # "Min Rect"
  # "Tracked targets"
  # "Best Pose"
  # "Alt Pose"
  # "Alt Pose"
  # "Pose"
  # "Alt Pose"
  # "Last Pose"
  # "RobotToCam"
  # "Det Corn"
  # "Min Rect"
  # "Pose"
  # "Detect Corn"
  # "Min Rect"
  # "Tracked targets"
  # "Make field"
  # "Best Pose"
  # "Alt Pose"
  # "Alt Pose"
  # "Pose"
  # "Alt Pose"
  n1 = call <vilib>:"TargetCorner_New.vi"("Y"=w413, "X"=w412) -> ("TargetCorner"=w405:T7)  [unwired: 9 in]
  n2 = call <vilib>:"TargetCorner_New.vi"("Y"=w411, "X"=w410) -> ("TargetCorner"=w404:T7)  [unwired: 9 in]
  n3 = call <vilib>:"TargetCorner_New.vi"("Y"=w409, "X"=w408) -> ("TargetCorner"=w403:T7)  [unwired: 9 in]
  n4 = call <vilib>:"TargetCorner_New.vi"("Y"=w401, "X"=w400) -> ("TargetCorner"=w393:T7)  [unwired: 9 in]
  n5 = call <vilib>:"TargetCorner_New.vi"("Y"=w399, "X"=w398) -> ("TargetCorner"=w392:T7)  [unwired: 9 in]
  n6 = call <vilib>:"TargetCorner_New.vi"("Y"=w407, "X"=w406) -> ("TargetCorner"=w402:T7)  [unwired: 9 in]
  n7 = call <vilib>:"TargetCorner_New.vi"("Y"=w397, "X"=w396) -> ("TargetCorner"=w391:T7)  [unwired: 9 in]
  n8 = call <vilib>:"TargetCorner_New.vi"("Y"=w395, "X"=w394) -> ("TargetCorner"=w390:T7)  [unwired: 9 in]
  n9 = call <vilib>:"Translation3d_Create.vi"("Z"=w387, "Y"=w385, "X"=w386) -> ("TRANSLATION3D"=w381:T3)  [unwired: 8 in]
  n10 = call <vilib>:"Translation3d_Create.vi"("Z"=w379, "Y"=w377, "X"=w378) -> ("TRANSLATION3D"=w373:T3)  [unwired: 8 in]
  n11 = call <vilib>:"TargetCorner_New.vi"("Y"=w363, "X"=w362) -> ("TargetCorner"=w355:T7)  [unwired: 9 in]
  n12 = call <vilib>:"TargetCorner_New.vi"("Y"=w361, "X"=w360) -> ("TargetCorner"=w354:T7)  [unwired: 9 in]
  n13 = call <vilib>:"TargetCorner_New.vi"("Y"=w359, "X"=w358) -> ("TargetCorner"=w353:T7)  [unwired: 9 in]
  n14 = call <vilib>:"TargetCorner_New.vi"("Y"=w351, "X"=w350) -> ("TargetCorner"=w343:T7)  [unwired: 9 in]
  n15 = call <vilib>:"TargetCorner_New.vi"("Y"=w313, "X"=w312) -> ("TargetCorner"=w305:T7)  [unwired: 9 in]
  n16 = call <vilib>:"TargetCorner_New.vi"("Y"=w349, "X"=w348) -> ("TargetCorner"=w342:T7)  [unwired: 9 in]
  n17 = call <vilib>:"TargetCorner_New.vi"("Y"=w311, "X"=w310) -> ("TargetCorner"=w304:T7)  [unwired: 9 in]
  n18 = call <vilib>:"TargetCorner_New.vi"("Y"=w357, "X"=w356) -> ("TargetCorner"=w352:T7)  [unwired: 9 in]
  n19 = call <vilib>:"TargetCorner_New.vi"("Y"=w347, "X"=w346) -> ("TargetCorner"=w341:T7)  [unwired: 9 in]
  n20 = call <vilib>:"TargetCorner_New.vi"("Y"=w309, "X"=w308) -> ("TargetCorner"=w303:T7)  [unwired: 9 in]
  n21 = call <vilib>:"Translation3d_Create.vi"("Z"=w337, "Y"=w335, "X"=w336) -> ("TRANSLATION3D"=w331:T3)  [unwired: 8 in]
  n22 = call <vilib>:"TargetCorner_New.vi"("Y"=w301, "X"=w300) -> ("TargetCorner"=w293:T7)  [unwired: 9 in]
  n23 = call <vilib>:"Rotation3d_Create_RollPitchYaw.vi"("Yaw"=w374, "Pitch"=w375, "Roll"=w376) -> ("Rotation3d"=w372:T4)  [unwired: 8 in]
  n24 = call <vilib>:"TargetCorner_New.vi"("Y"=w299, "X"=w298) -> ("TargetCorner"=w292:T7)  [unwired: 9 in]
  n25 = call <vilib>:"Rotation3d_Create_RollPitchYaw.vi"("Yaw"=w382, "Pitch"=w383, "Roll"=w384) -> ("Rotation3d"=w380:T4)  [unwired: 8 in]
  n26 = call <vilib>:"Translation3d_Create.vi"("Z"=w329, "Y"=w327, "X"=w328) -> ("TRANSLATION3D"=w323:T3)  [unwired: 8 in]
  n27 = call <vilib>:"TargetCorner_New.vi"("Y"=w345, "X"=w344) -> ("TargetCorner"=w340:T7)  [unwired: 9 in]
  n28 = call <vilib>:"TargetCorner_New.vi"("Y"=w307, "X"=w306) -> ("TargetCorner"=w302:T7)  [unwired: 9 in]
  n29 = call <vilib>:"TargetCorner_New.vi"("Y"=w297, "X"=w296) -> ("TargetCorner"=w291:T7)  [unwired: 9 in]
  n30 = call <vilib>:"Translation3d_Create.vi"("Z"=w279, "Y"=w277, "X"=w278) -> ("TRANSLATION3D"=w273:T3)  [unwired: 8 in]
  n31 = call <vilib>:"TargetCorner_New.vi"("Y"=w295, "X"=w294) -> ("TargetCorner"=w290:T7)  [unwired: 9 in]
  n32 = call <vilib>:"Translation3d_Create.vi"("Z"=w287, "Y"=w285, "X"=w286) -> ("TRANSLATION3D"=w281:T3)  [unwired: 8 in]
  n33 = call <vilib>:"Rotation3d_Create_RollPitchYaw.vi"("Yaw"=w332, "Pitch"=w333, "Roll"=w334) -> ("Rotation3d"=w330:T4)  [unwired: 8 in]
  n34 = call <vilib>:"Rotation3d_Create_RollPitchYaw.vi"("Yaw"=w324, "Pitch"=w325, "Roll"=w326) -> ("Rotation3d"=w322:T4)  [unwired: 8 in]
  n35 = call "test_PhotonPoseEstimator_Common_Make_Field.vi"() -> ("AprilTagFieldLayout"=w26:T10)  [unwired: 11 in]
  n36 = call <vilib>:"Rotation3d_Create_RollPitchYaw.vi"("Yaw"=w274, "Pitch"=w275, "Roll"=w276) -> ("Rotation3d"=w272:T4)  [unwired: 8 in]
  n37 = call <vilib>:"TargetCorner_New.vi"("Y"=w227, "X"=w226) -> ("TargetCorner"=w219:T7)  [unwired: 9 in]
  n38 = call <vilib>:"Rotation3d_Create_RollPitchYaw.vi"("Yaw"=w282, "Pitch"=w283, "Roll"=w284) -> ("Rotation3d"=w280:T4)  [unwired: 8 in]
  n39 = call <vilib>:"TargetCorner_New.vi"("Y"=w225, "X"=w224) -> ("TargetCorner"=w218:T7)  [unwired: 9 in]
  n40 = call <vilib>:"TargetCorner_New.vi"("Y"=w223, "X"=w222) -> ("TargetCorner"=w217:T7)  [unwired: 9 in]
  n41 = call <vilib>:"TargetCorner_New.vi"("Y"=w215, "X"=w214) -> ("TargetCorner"=w207:T7)  [unwired: 9 in]
  n42 = call <vilib>:"TargetCorner_New.vi"("Y"=w213, "X"=w212) -> ("TargetCorner"=w206:T7)  [unwired: 9 in]
  n43 = call <vilib>:"TargetCorner_New.vi"("Y"=w221, "X"=w220) -> ("TargetCorner"=w216:T7)  [unwired: 9 in]
  n44 = call <vilib>:"TargetCorner_New.vi"("Y"=w211, "X"=w210) -> ("TargetCorner"=w205:T7)  [unwired: 9 in]
  n45 = call <vilib>:"TargetCorner_New.vi"("Y"=w209, "X"=w208) -> ("TargetCorner"=w204:T7)  [unwired: 9 in]
  n46 = call <vilib>:"Translation3d_Create.vi"("Z"=w201, "Y"=w199, "X"=w200) -> ("TRANSLATION3D"=w195:T3)  [unwired: 8 in]
  n47 = call <vilib>:"Translation3d_Create.vi"("Z"=w193, "Y"=w191, "X"=w192) -> ("TRANSLATION3D"=w187:T3)  [unwired: 8 in]
  n48 = Build Array(w405, w404, w403, w402) -> (w389:T7[])
  n49 = Build Array(w393, w392, w391, w390) -> (w388:T7[])
  n50 = call <vilib>:"TargetCorner_New.vi"("Y"=w178, "X"=w177) -> ("TargetCorner"=w170:T7)  [unwired: 9 in]
  n51 = call <vilib>:"TargetCorner_New.vi"("Y"=w176, "X"=w175) -> ("TargetCorner"=w169:T7)  [unwired: 9 in]
  n52 = call <vilib>:"TargetCorner_New.vi"("Y"=w174, "X"=w173) -> ("TargetCorner"=w168:T7)  [unwired: 9 in]
  n53 = call <vilib>:"TargetCorner_New.vi"("Y"=w166, "X"=w165) -> ("TargetCorner"=w158:T7)  [unwired: 9 in]
  n54 = call <vilib>:"TargetCorner_New.vi"("Y"=w128, "X"=w127) -> ("TargetCorner"=w120:T7)  [unwired: 9 in]
  n55 = call <vilib>:"TargetCorner_New.vi"("Y"=w164, "X"=w163) -> ("TargetCorner"=w157:T7)  [unwired: 9 in]
  n56 = call <vilib>:"TargetCorner_New.vi"("Y"=w126, "X"=w125) -> ("TargetCorner"=w119:T7)  [unwired: 9 in]
  n57 = call <vilib>:"TargetCorner_New.vi"("Y"=w172, "X"=w171) -> ("TargetCorner"=w167:T7)  [unwired: 9 in]
  n58 = call <vilib>:"TargetCorner_New.vi"("Y"=w162, "X"=w161) -> ("TargetCorner"=w156:T7)  [unwired: 9 in]
  n59 = call <vilib>:"TargetCorner_New.vi"("Y"=w124, "X"=w123) -> ("TargetCorner"=w118:T7)  [unwired: 9 in]
  n60 = call <vilib>:"Translation3d_Create.vi"("Z"=w152, "Y"=w150, "X"=w151) -> ("TRANSLATION3D"=w146:T3)  [unwired: 8 in]
  n61 = call <vilib>:"TargetCorner_New.vi"("Y"=w116, "X"=w115) -> ("TargetCorner"=w108:T7)  [unwired: 9 in]
  n62 = call <vilib>:"Rotation3d_Create_RollPitchYaw.vi"("Yaw"=w188, "Pitch"=w189, "Roll"=w190) -> ("Rotation3d"=w186:T4)  [unwired: 8 in]
  n63 = call <vilib>:"TargetCorner_New.vi"("Y"=w114, "X"=w113) -> ("TargetCorner"=w107:T7)  [unwired: 9 in]
  n64 = call <vilib>:"Rotation3d_Create_RollPitchYaw.vi"("Yaw"=w196, "Pitch"=w197, "Roll"=w198) -> ("Rotation3d"=w194:T4)  [unwired: 8 in]
  n65 = call <vilib>:"Translation3d_Create.vi"("Z"=w144, "Y"=w142, "X"=w143) -> ("TRANSLATION3D"=w138:T3)  [unwired: 8 in]
  n66 = call <vilib>:"TargetCorner_New.vi"("Y"=w160, "X"=w159) -> ("TargetCorner"=w155:T7)  [unwired: 9 in]
  n67 = call <vilib>:"TargetCorner_New.vi"("Y"=w122, "X"=w121) -> ("TargetCorner"=w117:T7)  [unwired: 9 in]
  n68 = call <vilib>:"TargetCorner_New.vi"("Y"=w112, "X"=w111) -> ("TargetCorner"=w106:T7)  [unwired: 9 in]
  n69 = call <vilib>:"Translation3d_Create.vi"("Z"=w94, "Y"=w92, "X"=w93) -> ("TRANSLATION3D"=w88:T3)  [unwired: 8 in]
  n70 = call <vilib>:"Transform3d_Create_Trans3dRot3d.vi"("Rotation3d"=w380, "Translation3d"=w381) -> ("Transform3d"=w370:T8)  [unwired: 9 in]
  n71 = call <vilib>:"TargetCorner_New.vi"("Y"=w110, "X"=w109) -> ("TargetCorner"=w105:T7)  [unwired: 9 in]
  n72 = call <vilib>:"Transform3d_Create_Trans3dRot3d.vi"("Rotation3d"=w372, "Translation3d"=w373) -> ("Transform3d"=w371:T8)  [unwired: 9 in]
  n73 = Build Array(w355, w354, w353, w352) -> (w339:T7[])
  n74 = call <vilib>:"Translation3d_Create.vi"("Z"=w102, "Y"=w100, "X"=w101) -> ("TRANSLATION3D"=w96:T3)  [unwired: 8 in]
  n75 = Build Array(w343, w342, w341, w340) -> (w338:T7[])
  n76 = Build Array(w305, w304, w303, w302) -> (w289:T7[])
  n77 = Build Array(w293, w292, w291, w290) -> (w288:T7[])
  n78 = call <vilib>:"Rotation3d_Create_RollPitchYaw.vi"("Yaw"=w147, "Pitch"=w148, "Roll"=w149) -> ("Rotation3d"=w145:T4)  [unwired: 8 in]
  n79 = call <vilib>:"Rotation3d_Create_RollPitchYaw.vi"("Yaw"=w139, "Pitch"=w140, "Roll"=w141) -> ("Rotation3d"=w137:T4)  [unwired: 8 in]
  n80 = call <vilib>:"Transform3d_Create_Trans3dRot3d.vi"("Rotation3d"=w330, "Translation3d"=w331) -> ("Transform3d"=w320:T8)  [unwired: 9 in]
  n81 = call <vilib>:"Rotation3d_Create_RollPitchYaw.vi"("Yaw"=w89, "Pitch"=w90, "Roll"=w91) -> ("Rotation3d"=w87:T4)  [unwired: 8 in]
  n82 = call <vilib>:"Transform3d_Create_Trans3dRot3d.vi"("Rotation3d"=w322, "Translation3d"=w323) -> ("Transform3d"=w321:T8)  [unwired: 9 in]
  n83 = call <vilib>:"Transform3d_Create_Trans3dRot3d.vi"("Rotation3d"=w272, "Translation3d"=w273) -> ("Transform3d"=w271:T8)  [unwired: 9 in]
  n84 = call <vilib>:"Rotation3d_Create_RollPitchYaw.vi"("Yaw"=w97, "Pitch"=w98, "Roll"=w99) -> ("Rotation3d"=w95:T4)  [unwired: 8 in]
  n85 = call <vilib>:"Transform3d_Create_Trans3dRot3d.vi"("Rotation3d"=w280, "Translation3d"=w281) -> ("Transform3d"=w270:T8)  [unwired: 9 in]
  n86 = Build Array(w219, w218, w217, w216) -> (w203:T7[])
  n87 = Build Array(w207, w206, w205, w204) -> (w202:T7[])
  n88 = call <vilib>:"Transform3d_Create_Trans3dRot3d.vi"("Rotation3d"=w194, "Translation3d"=w195) -> ("Transform3d"=w185:T8)  [unwired: 9 in]
  n89 = call <vilib>:"Transform3d_Create_Trans3dRot3d.vi"("Rotation3d"=w186, "Translation3d"=w187) -> ("Transform3d"=w59:T8)  [unwired: 9 in]
  n90 = Build Array(w170, w169, w168, w167) -> (w154:T7[])
  n91 = Build Array(w158, w157, w156, w155) -> (w153:T7[])
  n92 = Build Array(w120, w119, w118, w117) -> (w104:T7[])
  n93 = Build Array(w108, w107, w106, w105) -> (w103:T7[])
  n94 = call <vilib>:"Transform3d_Create_Trans3dRot3d.vi"("Rotation3d"=w145, "Translation3d"=w146) -> ("Transform3d"=w135:T8)  [unwired: 9 in]
  n95 = call <vilib>:"PhotonTrackedTarget_New.vi"("Pitch"=w414, "Yaw"=w419, "Fiducial Id"=w417, "Area"=w415, "Skew"=w416, "ObjDetectId"=0, "DetectedCorners"=w388, "DetectObjConf"=sgl 0.0, "BestCameraToTarget"=w371, "AltCameraToTarget"=w370, "MinAreaRectCorners"=w389, "Pose Ambiguity"=w418) -> ("TrackedTarget"=w269:T6)  [unwired: 3 in]
  n96 = call <vilib>:"Transform3d_Create_Trans3dRot3d.vi"("Rotation3d"=w137, "Translation3d"=w138) -> ("Transform3d"=w136:T8)  [unwired: 9 in]
  n97 = call <vilib>:"Transform3d_Create_Trans3dRot3d.vi"("Rotation3d"=w87, "Translation3d"=w88) -> ("Transform3d"=w86:T8)  [unwired: 9 in]
  n98 = call <vilib>:"Transform3d_Create_Trans3dRot3d.vi"("Rotation3d"=w95, "Translation3d"=w96) -> ("Transform3d"=w85:T8)  [unwired: 9 in]
  n99 = call <vilib>:"PhotonTrackedTarget_New.vi"("Pitch"=w364, "Yaw"=w369, "Fiducial Id"=w367, "Area"=w365, "Skew"=w366, "ObjDetectId"=0, "DetectedCorners"=w338, "DetectObjConf"=sgl 0.0, "BestCameraToTarget"=w321, "AltCameraToTarget"=w320, "MinAreaRectCorners"=w339, "Pose Ambiguity"=w368) -> ("TrackedTarget"=w268:T6)  [unwired: 3 in]
  n100 = call <vilib>:"PhotonTrackedTarget_New.vi"("Pitch"=w314, "Yaw"=w319, "Fiducial Id"=w317, "Area"=w315, "Skew"=w316, "ObjDetectId"=0, "DetectedCorners"=w288, "DetectObjConf"=sgl 0.0, "BestCameraToTarget"=w271, "AltCameraToTarget"=w270, "MinAreaRectCorners"=w289, "Pose Ambiguity"=w318) -> ("TrackedTarget"=w267:T6)  [unwired: 3 in]
  n101 = call <vilib>:"PhotonTrackedTarget_New.vi"("Pitch"=w228, "Yaw"=w233, "Fiducial Id"=w231, "Area"=w229, "Skew"=w230, "ObjDetectId"=0, "DetectedCorners"=w202, "DetectObjConf"=sgl 0.0, "BestCameraToTarget"=w59, "AltCameraToTarget"=w185, "MinAreaRectCorners"=w203, "Pose Ambiguity"=w232) -> ("TrackedTarget"=w84:T6)  [unwired: 3 in]
  n102 = call <vilib>:"PhotonTrackedTarget_New.vi"("Pitch"=w179, "Yaw"=w184, "Fiducial Id"=w182, "Area"=w180, "Skew"=w181, "ObjDetectId"=0, "DetectedCorners"=w153, "DetectObjConf"=sgl 0.0, "BestCameraToTarget"=w136, "AltCameraToTarget"=w135, "MinAreaRectCorners"=w154, "Pose Ambiguity"=w183) -> ("TrackedTarget"=w83:T6)  [unwired: 3 in]
  n103 = call <vilib>:"PhotonTrackedTarget_New.vi"("Pitch"=w129, "Yaw"=w134, "Fiducial Id"=w132, "Area"=w130, "Skew"=w131, "ObjDetectId"=0, "DetectedCorners"=w103, "DetectObjConf"=sgl 0.0, "BestCameraToTarget"=w86, "AltCameraToTarget"=w85, "MinAreaRectCorners"=w104, "Pose Ambiguity"=w133) -> ("TrackedTarget"=w74:T6)  [unwired: 3 in]
  n104 = Build Array(w269, w268, w267) -> (w266:T6[])
  n105 = call <vilib>:"PhotonPipelineMetadata_New.vi"("TimeSinceLastPong"=w68, "SequenceID"=w67, "PublishTimestampMicros"=w66, "CaptureTimestampMicros"=w65) -> ("PhotonPipelineMetadata"=w64:T13)  [unwired: 7 in]
  n106 = Build Array(w84, w83, w74) -> (w82:T6[])
  n107 = call <vilib>:"PhotonPipelineResult_New.vi"("TrackedTargets"=w266, "Metadata"=w64) -> ("PhotonPipelineResult"=w265:T14)  [unwired: 9 in]
  n108 = call <vilib>:"PhotonPipelineMetadata_New.vi"("TimeSinceLastPong"=w73, "SequenceID"=w72, "PublishTimestampMicros"=w71, "CaptureTimestampMicros"=w70) -> ("PhotonPipelineMetadata"=w69:T13)  [unwired: 7 in]
  n109 = call <vilib>:"PhotonPipelineResult_New.vi"("TrackedTargets"=w82, "Metadata"=w69) -> ("PhotonPipelineResult"=w81:T14)  [unwired: 9 in]
  n110 = call <vilib>:"PhotonPipelineResult_SetTimeStampSecs.vi"("TimeStampSec"=1.0, "PhotonPipelineResult"=w265) -> ("Out PhotonPipelineResult"=w28:T14)  [unwired: 9 in]
  n111 = call <vilib>:"PhotonPipelineResult_SetTimeStampSecs.vi"("TimeStampSec"=7.0, "PhotonPipelineResult"=w81) -> ("Out PhotonPipelineResult"=w29:T14)  [unwired: 9 in]
  n112 = call <vilib>:"Translation3d_Create.vi"("Z"=w254, "Y"=w252, "X"=w253) -> ("TRANSLATION3D"=w248:T3)  [unwired: 8 in]
  n113 = call <vilib>:"Rotation3d_Create_RollPitchYaw.vi"("Yaw"=w249, "Pitch"=w250, "Roll"=w251) -> ("Rotation3d"=w247:T4)  [unwired: 8 in]
  n114 = call <vilib>:"Transform3d_Create_Trans3dRot3d.vi"("Rotation3d"=w247, "Translation3d"=w248) -> ("Transform3d"=w3:T8)  [unwired: 9 in]
  n115 = call <vilib>:"PhotonPoseEstimator_New.vi"("RobotToCamera"=w3, "Camera"=w5, "Strategy"=w4, "AprilTagFieldLayout"=w26) -> ("PhotonPoseEstimator"=w242:T17)  [unwired: 7 in]
  n116 = Build Array(w28, w29) -> (w27:T14[])
  n117 = call <vilib>:"Translation3d_Create.vi"("Z"=w241, "Y"=w239, "X"=w240) -> ("TRANSLATION3D"=w235:T3)  [unwired: 8 in]
  n118 = call <vilib>:"Rotation3d_Create_RollPitchYaw.vi"("Yaw"=w236, "Pitch"=w237, "Roll"=w238) -> ("Rotation3d"=w234:T4)  [unwired: 8 in]
  n119 = call <vilib>:"Pose3d_New_Trans3dRot3d.vi"("Rotation3d"=w234, "Translation3d"=w235) -> ("outPose3d"=w1:T2)  [unwired: 9 in]
  n120 = call <vilib>:"PhotonPoseEstimator_PackConfig.vi"("Initial Pose"=w1, "RobotToCamera"=w3, "HighestAmbiguity"=w6, "PirmaryStrategy"=w4, "Camera"=w5) -> ("PoseEstimator_Configuration"=w25:T19)  [unwired: 6 in]
  n121 = for {
    tunnel: w27 -> [w430] mode=indexing
    tunnel: w26 -> [w429]
    tunnel: w25 -> [w428]
    tunnel: [w426] -> w8
    n122 = call <vilib>:"PhotonPoseEstimator_Execute_ClosestToLastPose.vi"("Configuration"=w428, "AprilTagFieldLayout"=w429, "PIpeline Has \nNew Results"=TRUE ("PIpeline Has \nNew Results"), "PipelineResult"=w430) -> ("PhotonEstimatedRobotPose"=w426:T1)  [unwired: 2 in, 5 out]
  }
  n123 = call <vilib>:"PhotonPoseEstimator_SetLastPose.vi"("LastPose"=w1, "PhotonPoseEstimator"=w242) -> ("out PhotonPoseEstimator"=w49:T17)  [unwired: 9 in]
  n124 = call <vilib>:"PhotonPoseEstimator_SetHighestAmbiguity.vi"("HighestAmbiguity"=w6, "PhotonPoseEstimator"=w49) -> ("out PhotonPoseEstimator"=w50:T17)  [unwired: 9 in]
  n125 = call <vilib>:"PhotonPoseEstimator_Update_PipeResult.vi"("Has Results"=TRUE, "PipelineResult"=w28, "PhotonPoseEstimator"=w50) -> ("Pos Found"=→"1st Pos Found":bool, "PhotonEstimatedRobotPose"=→"1st Pose Est":T1, "out PhotonPoseEstimator"=w48:T17)  [unwired: 6 in]
  n126 = call <vilib>:"PhotonPoseEstimator_Update_PipeResult.vi"("Has Results"=w47, "PipelineResult"=w29, "PhotonPoseEstimator"=w48) -> ("Pos Found"=→"2nd Pos Found":bool, "PhotonEstimatedRobotPose"=w78:T1)  [unwired: 6 in, 1 out]
  "2nd Pose Est" <- w78
  n127 = call <vilib>:"PhotonPoseEstimator_Update_ClosestToLastPose.vi"("Has Results"=w47, "PipelineResult"=w29, "PhotonPoseEstimator"=w48) -> ("PhotonEstimatedRobotPose"=w2:T1)  [unwired: 6 in, 2 out]
  n128 = Unbundle By Name(w2) -> ("TimeStamp_Seconds"=w31:dbl, "EstimatedPose.Translation3d.X"=w37:dbl, "EstimatedPose.Translation3d.Y"=w36:dbl, "EstimatedPose.Translation3d.Z"=w35:dbl)
  n129 = Unbundle By Name(w78) -> ("TimeStamp_Seconds"=w243:dbl, "EstimatedPose.Translation3d.X"=w257:dbl, "EstimatedPose.Translation3d.Y"=w256:dbl, "EstimatedPose.Translation3d.Z"=w255:dbl)
  n130 = Unbundle By Name(w8) -> ("TimeStamp_Seconds"=w9:dbl, "EstimatedPose.Translation3d.X"=w15:dbl, "EstimatedPose.Translation3d.Y"=w14:dbl, "EstimatedPose.Translation3d.Z"=w13:dbl)
  n131 = call <vilib>:"Util_ApproxEquals.vi"("Tolerance"=0.01, "Value 2"=7.0, "Value 1"=w31) -> ("ApproxEquals"=w32:bool)  [unwired: 8 in]
  n132 = call <vilib>:"Util_ApproxEquals.vi"("Tolerance"=0.01, "Value 2"=7.0, "Value 1"=w243) -> ("ApproxEquals"=w244:bool)  [unwired: 8 in]
  n133 = call <vilib>:"Util_ApproxEquals.vi"("Tolerance"=0.01, "Value 2"=1.1, "Value 1"=w36) -> ("ApproxEquals"=w39:bool)  [unwired: 8 in]
  n134 = call <vilib>:"Util_ApproxEquals.vi"("Tolerance"=0.01, "Value 2"=0.9, "Value 1"=w37) -> ("ApproxEquals"=w44:bool)  [unwired: 8 in]
  n135 = call <vilib>:"Util_ApproxEquals.vi"("Tolerance"=0.01, "Value 2"=1.1, "Value 1"=w256) -> ("ApproxEquals"=w259:bool)  [unwired: 8 in]
  n136 = call <vilib>:"Util_ApproxEquals.vi"("Tolerance"=0.01, "Value 2"=0.9, "Value 1"=w257) -> ("ApproxEquals"=w422:bool)  [unwired: 8 in]
  n137 = call <vilib>:"Util_ApproxEquals.vi"("Tolerance"=0.01, "Value 2"=1.0, "Value 1"=w35) -> ("ApproxEquals"=w38:bool)  [unwired: 8 in]
  n138 = call <vilib>:"Util_ApproxEquals.vi"("Tolerance"=0.01, "Value 2"=7.0, "Value 1"=w9) -> ("ApproxEquals"=w10:bool)  [unwired: 8 in]
  n139 = call <vilib>:"Util_ApproxEquals.vi"("Tolerance"=0.01, "Value 2"=1.0, "Value 1"=w255) -> ("ApproxEquals"=w258:bool)  [unwired: 8 in]
  n140 = call <vilib>:"Util_ApproxEquals.vi"("Tolerance"=0.01, "Value 2"=1.1, "Value 1"=w14) -> ("ApproxEquals"=w17:bool)  [unwired: 8 in]
  n141 = call <vilib>:"Util_ApproxEquals.vi"("Tolerance"=0.01, "Value 2"=0.9, "Value 1"=w15) -> ("ApproxEquals"=w22:bool)  [unwired: 8 in]
  n142 = call <vilib>:"Util_ApproxEquals.vi"("Tolerance"=0.01, "Value 2"=1.0, "Value 1"=w13) -> ("ApproxEquals"=w16:bool)  [unwired: 8 in]
  n143 = Compound Arithmetic op=AND(w32, w44, w39, w38) -> (w30:bool)
  "Test 1 Passed" <- w30
  n144 = Compound Arithmetic op=AND(w244, w422, w259, w258) -> (w420:bool)
  "Test 0 Passed" <- w420
  n145 = Compound Arithmetic op=AND(w10, w22, w17, w16) -> (w7:bool)
  "Test 2 Passed" <- w7
  n146 = Compound Arithmetic op=AND(w420, w30, w7) -> (→"Test Passed":bool)
  "error out" <- "error in (no error)"
